vi "Load Config.vi"(8 "error in (no error)":errorcluster, 11 "DAQmxVoltageChannel in":refnum<class "VoltageInChannel.lvclass">) -> (0 "error out":errorcluster, 3 "DAQmxVoltageChannel out":refnum<class "VoltageInChannel.lvclass">)   [LabVIEW 2020, in "VolatusDAQConfig.lvlib" / "VoltageInChannel.lvclass"]
uses:
  VoltageInChannel.lvclass
  C:/dev/lv20CE/relink/lv-volatus/VolatusConfig/VolatusConfigElement/VolatusConfigElement.lvclass
  VolatusConfig/VolatusConfigElement/VolatusConfigElement.lvclass/VolatusConfigElement.ctl
  VoltageInChannel.lvclass/VoltageInChannel.ctl
  VolatusConfig/VolatusConfigElement/Element.vi
  VolatusConfig/VolatusConfigElement/VolatusConfigElement.lvclass
  lv-cdm/CDM-Config/Config Element/Config Element.lvclass
  C:/dev/lv20CE/relink/lv-volatus/VolatusDAQConfig/DAQmxChannel/DAQmxChannel.lvclass
  C:/dev/lv20CE/relink/lv-volatus/VolatusConfig/Channel/Channel.lvclass
  C:/dev/lv20CE/relink/lv-volatus/VolatusDAQConfig/DAQmxVoltageChannel/VoltageInChannel.lvclass
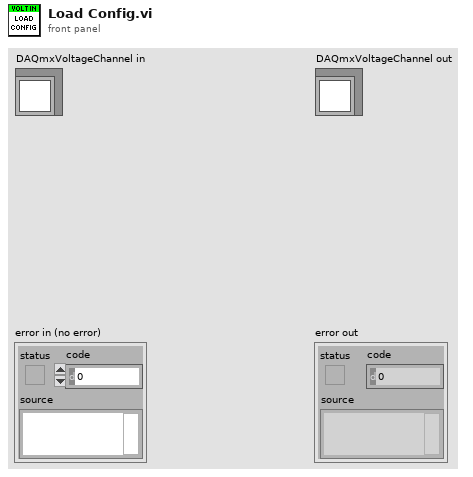
[diagram p1: front panel]
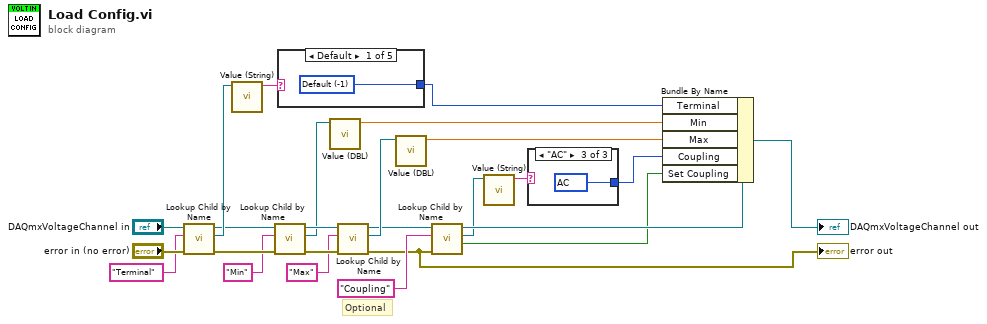
[diagram p0: block diagram]
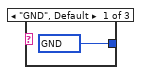
[diagram p2: hidden frame]
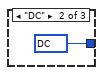
[diagram p3: hidden frame]
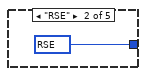
[diagram p4: hidden frame]
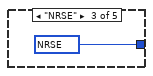
[diagram p5: hidden frame]
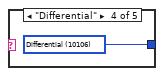
[diagram p6: hidden frame]
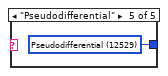
[diagram p7: hidden frame]
diagram:
  # "Optional"
  n1 = call "Lookup Child by Name.vi"("error in (no error)"="error in (no error)", "Child Name"="Terminal", "VolatusConfigElement in"="DAQmxVoltageChannel in") -> ("error out"=w24:errorcluster, "Child"=w21:refnum<class "Config Element.lvclass">, "VolatusConfigElement out"=w16:refnum<class "VoltageInChannel.lvclass">)  [unwired: 5 in, 1 out]
  n2 = call "Value (String).vi"("Config Element in"=w21) -> ("String Value"=w20:string)  [unwired: 9 in, 1 out]
  n3 = call "Lookup Child by Name.vi"("error in (no error)"=w24, "Child Name"="Min", "VolatusConfigElement in"=w16) -> ("error out"=w17:errorcluster, "Child"=w13:refnum<class "Config Element.lvclass">, "VolatusConfigElement out"=w15:refnum<class "VoltageInChannel.lvclass">)  [unwired: 5 in, 1 out]
  n4 = case shown="Default" w20 {
    tunnel: [w26 w27 w28 w29 w30] -> w19
    frame Default {
      w26 = -1 items=["Default"=-1, "RSE"=10083, "NRSE"=10078, "Differential"=10106, "Pseudodifferential"=12529] ("input terminal configuration")
    }
    frame "RSE" {
      w27 = 10083 items=["Default"=-1, "RSE"=10083, "NRSE"=10078, "Differential"=10106, "Pseudodifferential"=12529] ("input terminal configuration")
    }
    frame "NRSE" {
      w28 = 10078 items=["Default"=-1, "RSE"=10083, "NRSE"=10078, "Differential"=10106, "Pseudodifferential"=12529] ("input terminal configuration")
    }
    frame "Differential" {
      w29 = 10106 items=["Default"=-1, "RSE"=10083, "NRSE"=10078, "Differential"=10106, "Pseudodifferential"=12529] ("input terminal configuration")
    }
    frame "Pseudodifferential" {
      w30 = 12529 items=["Default"=-1, "RSE"=10083, "NRSE"=10078, "Differential"=10106, "Pseudodifferential"=12529] ("input terminal configuration")
    }
  }
  n5 = call "Value (DBL).vi"("Config Element in"=w13) -> ("DBL Value"=w12:dbl)  [unwired: 9 in, 1 out]
  n6 = call "Lookup Child by Name.vi"("error in (no error)"=w17, "Child Name"="Max", "VolatusConfigElement in"=w15) -> ("error out"=w4:errorcluster, "Child"=w11:refnum<class "Config Element.lvclass">, "VolatusConfigElement out"=w8:refnum<class "VoltageInChannel.lvclass">)  [unwired: 5 in, 1 out]
  "error out" <- w4
  n7 = call "Value (DBL).vi"("Config Element in"=w11) -> ("DBL Value"=w10:dbl)  [unwired: 9 in, 1 out]
  n8 = call "Lookup Child by Name.vi"("error in (no error)"=w4, "Child Name"="Coupling", "VolatusConfigElement in"=w8) -> ("Found"=w1:bool, "Child"=w5:refnum<class "Config Element.lvclass">, "VolatusConfigElement out"=w6:refnum<class "VoltageInChannel.lvclass">)  [unwired: 5 in, 1 out]
  n9 = call "Value (String).vi"("Config Element in"=w5) -> ("String Value"=w3:string)  [unwired: 9 in, 1 out]
  n10 = case shown="\"AC\"" w3 {
    tunnel: [w31 w32 w33] -> w2
    frame "GND", Default {
      w31 = 10066 items=["AC"=10045, "DC"=10050, "GND"=10066] ("AI.Coupling")
    }
    frame "DC" {
      w32 = 10050 items=["AC"=10045, "DC"=10050, "GND"=10066] ("AI.Coupling")
    }
    frame "AC" {
      w33 = 10045 items=["AC"=10045, "DC"=10050, "GND"=10066] ("AI.Coupling")
    }
  }
  n11 = Bundle By Name(cluster=w6, "Terminal"=w19, "Min"=w12, "Max"=w10, "Coupling"=w2, "Set Coupling"=w1) -> (→"DAQmxVoltageChannel out":refnum<class "VoltageInChannel.lvclass">)
